vi "Test Case only Added to Suite once.vi"(8 "error in (no error)":errorcluster, 11 "Test Case In":refnum<class "LUnit Test Suite Tests.lvclass">) -> (0 "error out":errorcluster, 3 "Test Case Out":refnum<class "LUnit Test Suite Tests.lvclass">)   [LabVIEW 2020, in "LUnit Test Suite Tests.lvclass"]
uses:
  LUnit Test Suite Tests.lvclass
  LUnit Test Suite Tests.lvclass/LUnit Test Suite Tests.ctl
  source/LUnit Test Suite.lvclass
  b74e4934-f044-4222-b3dd-fc90e6c1bd4f.vi
  Test Doubles/Test Case Test Double Child/Light Test Case Double.lvclass
  C:/git/astemes-lunit/source/Core/Runnable/Runnable.lvclass
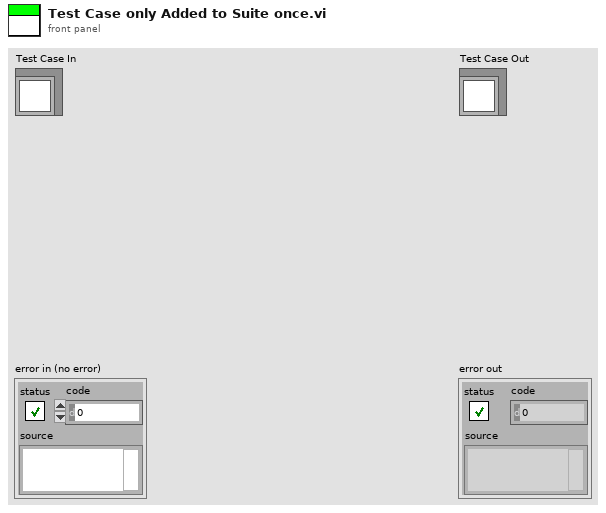
[diagram p1: front panel]
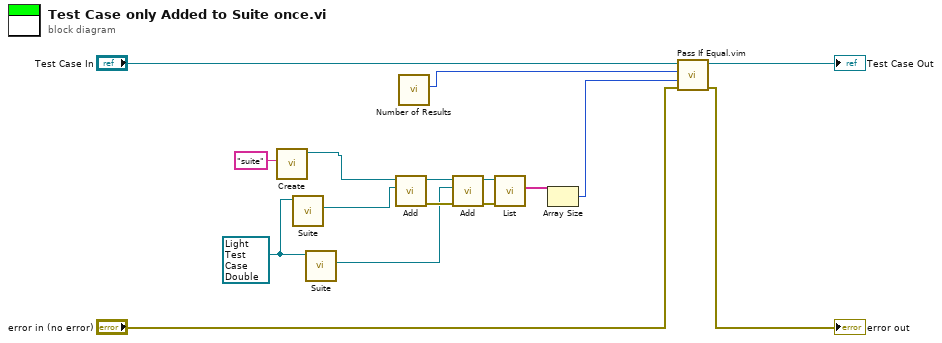
[diagram p0: block diagram]
diagram:
  w5 = refnum<class "Light Test Case Double.lvclass"> refnum ("Light Test Case Double.lvclass")
  n1 = call "Create.vi"("Suite Name"="suite") -> ("LUnit Test Suite Out"=w4:refnum<class "LUnit Test Suite.lvclass">)  [unwired: 9 in, 1 out]
  n2 = call-dynamic "Suite.vi"("LUnit Test Case In"=w5) -> ("LUnit Test Suite Out"=w6:refnum<class "LUnit Test Suite.lvclass">)  [unwired: 8 in, 2 out]
  n3 = call-dynamic "Suite.vi"("LUnit Test Case In"=w5) -> ("LUnit Test Suite Out"=w2:refnum<class "LUnit Test Suite.lvclass">)  [unwired: 8 in, 2 out]
  n4 = call "Add.vi"("Runnable"=w6, "LUnit Test Suite In"=w4) -> ("error out"=w8:errorcluster, "LUnit Test Suite Out"=w7:refnum<class "LUnit Test Suite.lvclass">)  [unwired: 8 in]
  n5 = call "Number of Results.vi"() -> ("number of methods"=w1:i32)  [unwired: 10 in, 1 out]
  n6 = call "Add.vi"("error in (no error)"=w8, "Runnable"=w2, "LUnit Test Suite In"=w7) -> ("error out"=w10:errorcluster, "LUnit Test Suite Out"=w9:refnum<class "LUnit Test Suite.lvclass">)  [unwired: 7 in]
  n7 = call "List.vi"("error in (no error)"=w10, "LUnit Test Suite In"=w9) -> ("List of Runnables"=w12:string[])  [unwired: 8 in, 1 out]
  n8 = Array Size(array=w12) -> (size(s)=w11:i32)
  n9 = call "Pass If Equal.vim"("error in (no error)"="error in (no error)", "Actual"=w11, "Expected"=w1, "LUnit Test Case In"="Test Case In") -> ("error out"=→"error out":errorcluster, "LUnit Test Case Out"=→"Test Case Out":refnum<class "LUnit Test Suite Tests.lvclass">)  [unwired: 6 in]
